vi "Get cif_can_writer_nixnet_CanMessage.vi"(8 "error in (no error)":errorcluster, 11 "gRPCid":T1) -> (0 "error out":errorcluster, 2 "package_templatemessage":T2, 3 "gRPCid out":T1)   [LabVIEW 2021, in "CanWriterNixnet_server.lvlib"]
uses:
  CanWriterNixnet_server.lvlib
  cif_can_writer_nixnet_CanMessage.ctl
  <vilib>/gRPC/LabVIEW gRPC Library/Shared/grpcId.ctl
  cif_can_writer_nixnet_CanMessage_Flat.ctl
  2ed25e12-861d-4677-8ead-ace2906b2041.vi
  <vilib>/gRPC/LabVIEW gRPC Library/Shared/TranslateGrpcError.vi
  <vilib>/gRPC/LabVIEW gRPC Library/Server API/Server/Get Server DLL Path.vi
  <vilib>/Utility/error.llb/Error Cluster From Error Code.vi
  <vilib>/gRPC/LabVIEW gRPC Library/grpc-lvsupport-release.lvlib
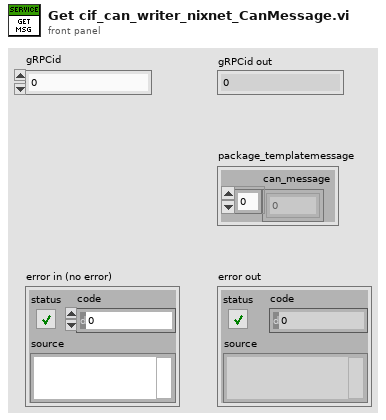
[diagram p1: front panel]
types:
  T1 = typedef "grpc-lvsupport-release.lvlib/grpcId.ctl" = u64
  T2 = typedef "CanWriterNixnet_server.lvlib/cif_can_writer_nixnet_CanMessage.ctl" = cluster{"can_message":u8[]}
  T3 = typedef "CanWriterNixnet_server.lvlib/cif_can_writer_nixnet_CanMessage_Flat.ctl" = cluster{"can_message":u8[]}
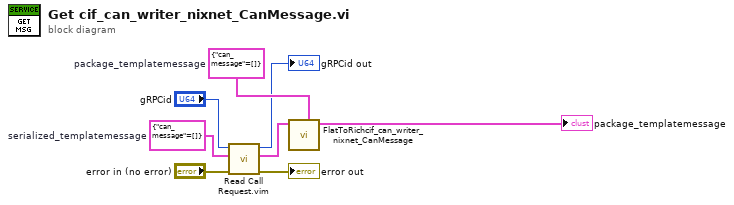
[diagram p0: block diagram]
diagram:
  w6 = T3 {"can_message"=[]}  # serialized_templatemessage
  w5 = T2 {"can_message"=[]}  # package_templatemessage
  n1 = call "Read Call Request.vim"("error in"="error in (no error)", "Request Type"=w6, "gRPCid in"="gRPCid") -> ("error out"=→"error out":errorcluster, "Request Data"=w4:T3, "gRPCid out"=→"gRPCid out":T1)  [unwired: 6 in]
  n2 = call "FlatToRichcif_can_writer_nixnet_CanMessage.vi"("OutputClusterType"=w5, "InputCluster"=w4) -> ("OutputCluster"=→"package_templatemessage":T2)  [unwired: 9 in]
